vi "DAQmx.Create AI Tasks.vi"(8 "error in":errorcluster, 11 "DAQmx in":refnum<class "DAQmx.lvclass">) -> (0 "error out":errorcluster, 3 "DAQmx out":refnum<class "DAQmx.lvclass">)   [LabVIEW 2019, in "DAQmx.lvclass"]
uses:
  DAQmx.lvclass
  typedefs/DAQ.Config.AI--Cluster--Array.ctl
  typedefs/DAQ.Config.AI--Cluster.ctl
  typedefs/DAQ.Config.AI.Coupling--enum.ctl
  typedefs/DAQ.Config.AI.Range--enum.ctl
  typedefs/DAQ.Config.Device Type--enum.ctl
  DAQmx.lvclass/DAQmx.ctl
  <vilib>/DAQmx/create/channels.llb/DAQmx Create Channel (AI-Voltage-Basic).vi
  <resource>/objmgr/daqmx.rc
panel:
  out "AI":T1 {"input terminal configuration" items=[""=-1, "Differential"=10106, "Pseudodifferential"=12529]; "Coupling" items=[""=0, "AC"=10045, "DC"=10050, "GND"=10066]}
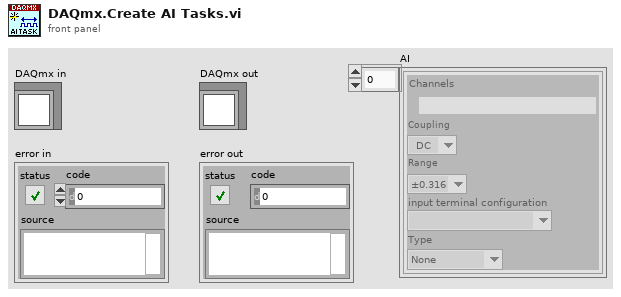
[diagram p1: front panel]
types:
  T1 = typedef "DAQmx.lvclass/DAQ.Config.AI--Cluster--Array.ctl" = T2[]
  T2 = typedef "DAQmx.lvclass/DAQ.Config.AI--Cluster.ctl" = cluster{"Channels":tag, "Coupling":T3, "Range":T4, "input terminal configuration":i32, "Type":T5}
  T3 = typedef "DAQmx.lvclass/DAQ.Config.AI.Coupling--enum.ctl" = u16
  T4 = typedef "DAQmx.lvclass/DAQ.Config.AI.Range--enum.ctl" = enum16{"±0.316", "±1.00", "±3.16", "±10.0", "±31.6", "±42.4", ""}
  T5 = typedef "DAQmx.lvclass/DAQ.Config.Device Type--enum.ctl" = enum16{"None", "USB-4431", "PXI-446x"}
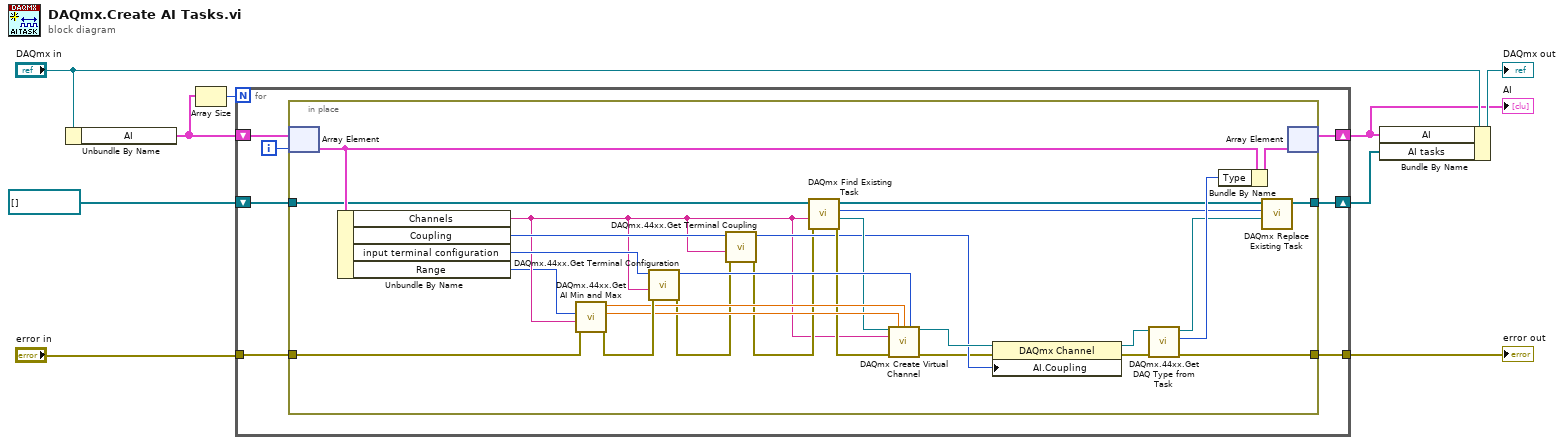
[diagram p0: block diagram]
diagram:
  n1 = Unbundle By Name("DAQmx in") -> ("AI"=w3:T1)
  n2 = Array Size(array=w3) -> (size(s)=w4:i32)
  n3 = for {
    N: w4 -> [_]
    tunnel: "error in" -> [w16]
    tunnel: [w13] -> w5
    shift-right: [w15] -> w2
    shift-left: refnum<k21>[] [] -> [w14]
    shift-right: [w10] -> w1
    shift-left: w3 -> [w12]
    i -> [w11]
    n4 = in-place {
      in-place-border: w16 -> [w43]
      in-place-border: [w41] -> w15
      in-place-border: w14 -> [w34]
      in-place-border: [w38] -> w13
      n5 = in-place-array #1(w12, w11) -> (w36:T2)
      n6 = Unbundle By Name(w36) -> ("Channels"=w18:tag, "Coupling"=w23:T3, "input terminal configuration"=w28:i32, "Range"=w17:T4)
      n7 = call "DAQmx.44xx.Get AI Min and Max.vi"("error in (no error)"=w43, "AI.channels"=w18, "AI.Range"=w17) -> ("error out"=w31:errorcluster, "AI.Max"=w30:dbl, "AI.Min"=w29:dbl)  [unwired: 6 in]
      n8 = call "DAQmx.44xx.Get Terminal Configuration.vi"("error in (no error)"=w31, "Channel in"=w18, "terminal configuration in"=w28) -> ("error out"=w20:errorcluster, "terminal configuration out"=w32:i32)  [unwired: 7 in]
      n9 = call "DAQmx.44xx.Get Terminal Coupling.vi"("error in (no error)"=w20, "Channel in"=w18, "Coupling in"=w23) -> ("error out"=w19:errorcluster, "AI.Coupling"=w22:i32)  [unwired: 7 in]
      n10 = call "DAQmx Find Existing Task.vi"("error in (no error)"=w19, "Channels"=w18, "Tasks in"=w34) -> ("error out"=w24:errorcluster, "Task out"=w25:refnum<k21>, "Task Index"=w27:i32, "Tasks out"=w26:refnum<k21>[])  [unwired: 5 in]
      n11 = call-poly <vilib>:"DAQmx Create Virtual Channel.vi"("task in"=w25, "maximum value"=w30, "minimum value"=w29, "input terminal configuration"=w32, "physical channels"=w18, "error in"=w24) -> ("task out"=w33:refnum<k21>, "error out"=w21:errorcluster)  [unwired: 8 in]
      n12 = property class="DAQmx Channel"(reference=w33, error in=w21, "AI.Coupling"=w22) -> (reference out=w37:refnum<k21>, error out=w40:errorcluster)
      n13 = call "DAQmx.44xx.Get DAQ Type from Task.vi"("error in (no error)"=w40, "Task in"=w37) -> ("error out"=w38:errorcluster, "DAQ Type"=w42:T5, "Task out"=w39:refnum<k21>)  [unwired: 5 in, 2 out]
      n14 = Bundle By Name(cluster=w36, "Type"=w42) -> (w35:T2)
      n15 = call "DAQmx Replace Existing Task.vi"("Task in"=w39, "Task Index"=w27, "Tasks in"=w26) -> ("Tasks out"=w41:refnum<k21>[])  [unwired: 8 in]
      n16 = in-place-array #1(w35) -> (w10:T1)  [unwired: 1 out]
    }
  }
  "error out" <- w5
  "AI" <- w1
  n17 = Bundle By Name(cluster="DAQmx in", "AI"=w1, "AI tasks"=w2) -> (→"DAQmx out":refnum<class "DAQmx.lvclass">)
